vi "toNextYear.vi"(7 "Values":i32[](array[numeric]), 11 "Cron in":T1) -> (3 "Cron out":T1)   [LabVIEW 2013, in "openCron.lvlib" / "Cron.lvclass"]
uses:
  Cron.lvclass
  CronTime -- cluster.ctl
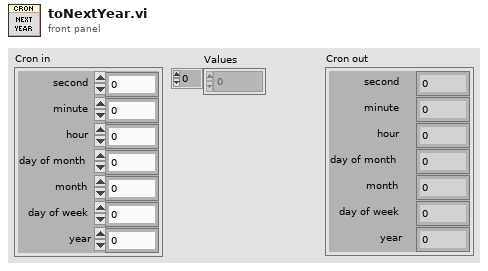
[diagram p1: front panel]
types:
  T1 = typedef "openCron.lvlib/Cron.lvclass/CronTime -- cluster.ctl" = cluster{"second":i32, "minute":i32, "hour":i32, "day of month":i32, "month":i32, "day of week":i32, "year":i32}
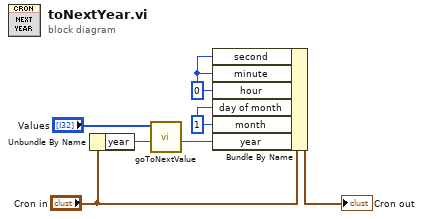
[diagram p0: block diagram]
diagram:
  w6 = 0 ("hour")
  w5 = 1 ("month")
  n1 = Unbundle By Name("Cron in") -> ("year"=w2:i32)
  n2 = call "goToNextValue.vi"("value in"=w2, "Values Pool"="Values") -> ("next value"=w1:i32)  [unwired: 8 in, 1 out]
  n3 = Bundle By Name(cluster="Cron in", "second"=w6, "minute"=w6, "hour"=w6, "day of month"=w5, "month"=w5, "year"=w1) -> (→"Cron out":T1)
